vi "PicoScopeospaGetValuesBulk.vi"(5 "Segment Range":T1 {"toSegmentIndex" format="%.4p"; "fromSegmentIndex" format="%.4p"}, 7 "Buffer and Transfer Settings":T2={"startIndex"=0, "Samples"=1000, "Down Sample Ratio"=1, "Down-Sample Mode"=1} {"Down-Sample Mode" items=["None"=2147483648, "Aggregate"=1, "Decimate"=2, "Average"=4]; "Down Sample Ratio" step=1; "Samples" format="%_6p"}, 8 "error in (no error)":errorcluster, 11 "handle in":i16) -> (0 "error out":errorcluster, 3 "handle out":i16, 4 "overflow":i16[](array[numeric]) format="%010b", 6 "noOfSamples":u64)   [LabVIEW 2010]
doc: "Calls GetValuesBulk"
uses:
  ps6000a.dll
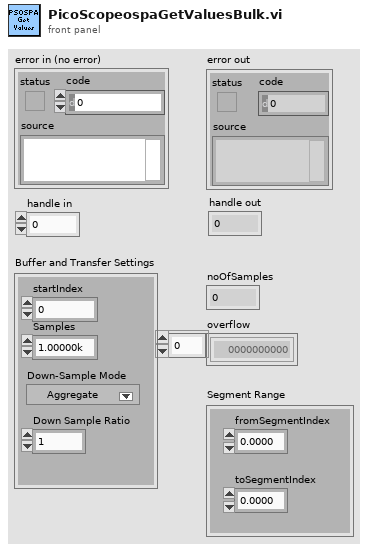
[diagram p1: front panel]
types:
  T1 = cluster{"fromSegmentIndex":u64, "toSegmentIndex":u64}
  T2 = cluster{"startIndex":u64, "Samples":u64, "Down Sample Ratio":u64, "Down-Sample Mode":u32}
  T3 = cluster{"status":bool, "code":u32, "source":string}
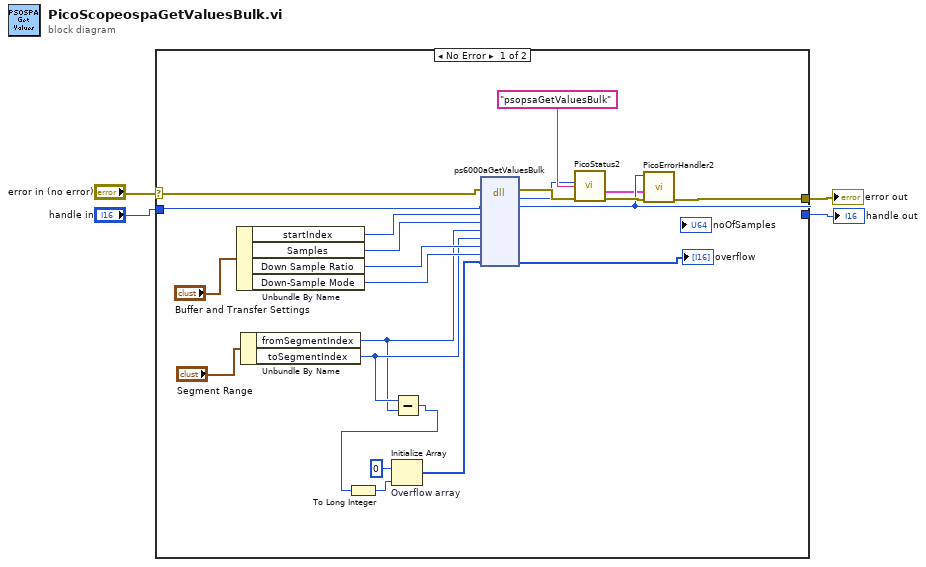
[diagram p0: block diagram]
diagram:
  n1 = case shown="No Error" "error in (no error)" {
    selector: "error in (no error)" -> [w9 w27]
    tunnel: "handle in" -> [w14 w28]
    tunnel: [w20 w28] -> w4
    tunnel: [w23 w27] -> w3
    frame No Error {
      n2 = Unbundle By Name("Buffer and Transfer Settings") -> ("startIndex"=w13:u64, "Samples"=w12:u64, "Down Sample Ratio"=w11:u64, "Down-Sample Mode"=w10:u32)
      n3 = Unbundle By Name("Segment Range") -> ("fromSegmentIndex"=w7:u64, "toSegmentIndex"=w8:u64)
      n4 = Subtract(x=w8, y=w7) -> (x-y=w15:u64)
      n5 = To Long Integer(number=w15) -> (32bit integer=w17:i32)
      n6 = Initialize Array "Overflow array"(i16 0 ("element"), w17) -> (w16:i16[])
      n7 = dll-call lib="ps6000a.dll" fn="ps6000aGetValuesBulk" ("ps3000.dll:_ps3000_open_unit@0")(error in=w9, "handle"=w14, "startIndex"=w13, "noOfSamples"=w12, "fromSegmentIndex"=w7, "toSegmentIndex"=w8, "downSampleRatio"=w11, "downSampleRatioMode"=w10, "overflow"=w16) -> (error out=w21:errorcluster, "PICO_STATUS"=w19:u32, "handle"=w20:i16, "overflow"=→"overflow":i16[])  [unwired: 8 in, 1 out]
      n8 = call "PicoStatus2.vi"("PICO source"="psopsaGetValuesBulk" ("source"), "Error in"=w21, "PICO STATUS"=w19) -> ("error out"=w26:errorcluster, "PICO_STATUS out"=w5:T3)  [unwired: 5 in]
      n9 = call "PicoErrorHandler2.vi"("error in (no error)"=w26, "PICO_STATUS in"=w5, "handle In"=w20) -> ("error out"=w23:errorcluster)  [unwired: 8 in]
    }
    frame Error {
    }
  }
  "error out" <- w3
  "handle out" <- w4
